vi "WLAN_FrameAnalysisV3.vi"(0 "input cluster":cluster{"t0":dbl, "dt":dbl, "Y":cdb[]}, 5 "error in (no error)":errorcluster) -> (3 "SNR dB":dbl, 8 "Modulation parameter LP":T1, 9 "outputbitsHP":i8[](array[numeric]), 10 "SIG valid?":bool, 11 "Frequency offset":dbl, 12 "SNR dB HP":dbl, 13 "SNR dB LP":dbl, 14 "output bits":i8[](array[numeric]), 16 "Modulation parameter":T1, 17 "Constellation":cdb[](graph), 19 "error out":errorcluster)   [LabVIEW 2022 SP3]
panel:
  in  "Expected message HP":string="Critical Dataaaaa\nCritical Dataaaaa\nCritical Dataaaaa\nCritical Dataaaaa\nCritical Dataaaaa"
  in  "Expected message LP":string="Non Critical Data\nNon Critical Data\nNon Critical Data\nNon Critical Data\nNon Critical Data"
  out "SNR Valid?":bool
  out "Noise Power":dbl
  out "Signal Power":dbl
  out "Alpha":u32
  out "subarray":cdb[](array[numeric])
  out "size(s) 6":i32
  out "size(s) 5":i32
  out "size(s) 4":i32
  out "x+y":dbl
  out "Frequency offset(LTF)":dbl
  out "Frequency offset corrected signal 2":cluster{"t0":dbl, "dt":dbl, "Y":dbl[]}(graph)
  out "size(s) 3":i32
  out "size(s) 2":i32
  out "size(s)":i32
  out "Symbol numbers":i32
  out "encoded bit numbers":u32
  out "original bit numbers":u32
  out "Channel Esitimate":dbl[](graph)
  out "Frequency offset corrected signal":cluster{"t0":dbl, "dt":dbl, "Y":dbl[]}(graph)
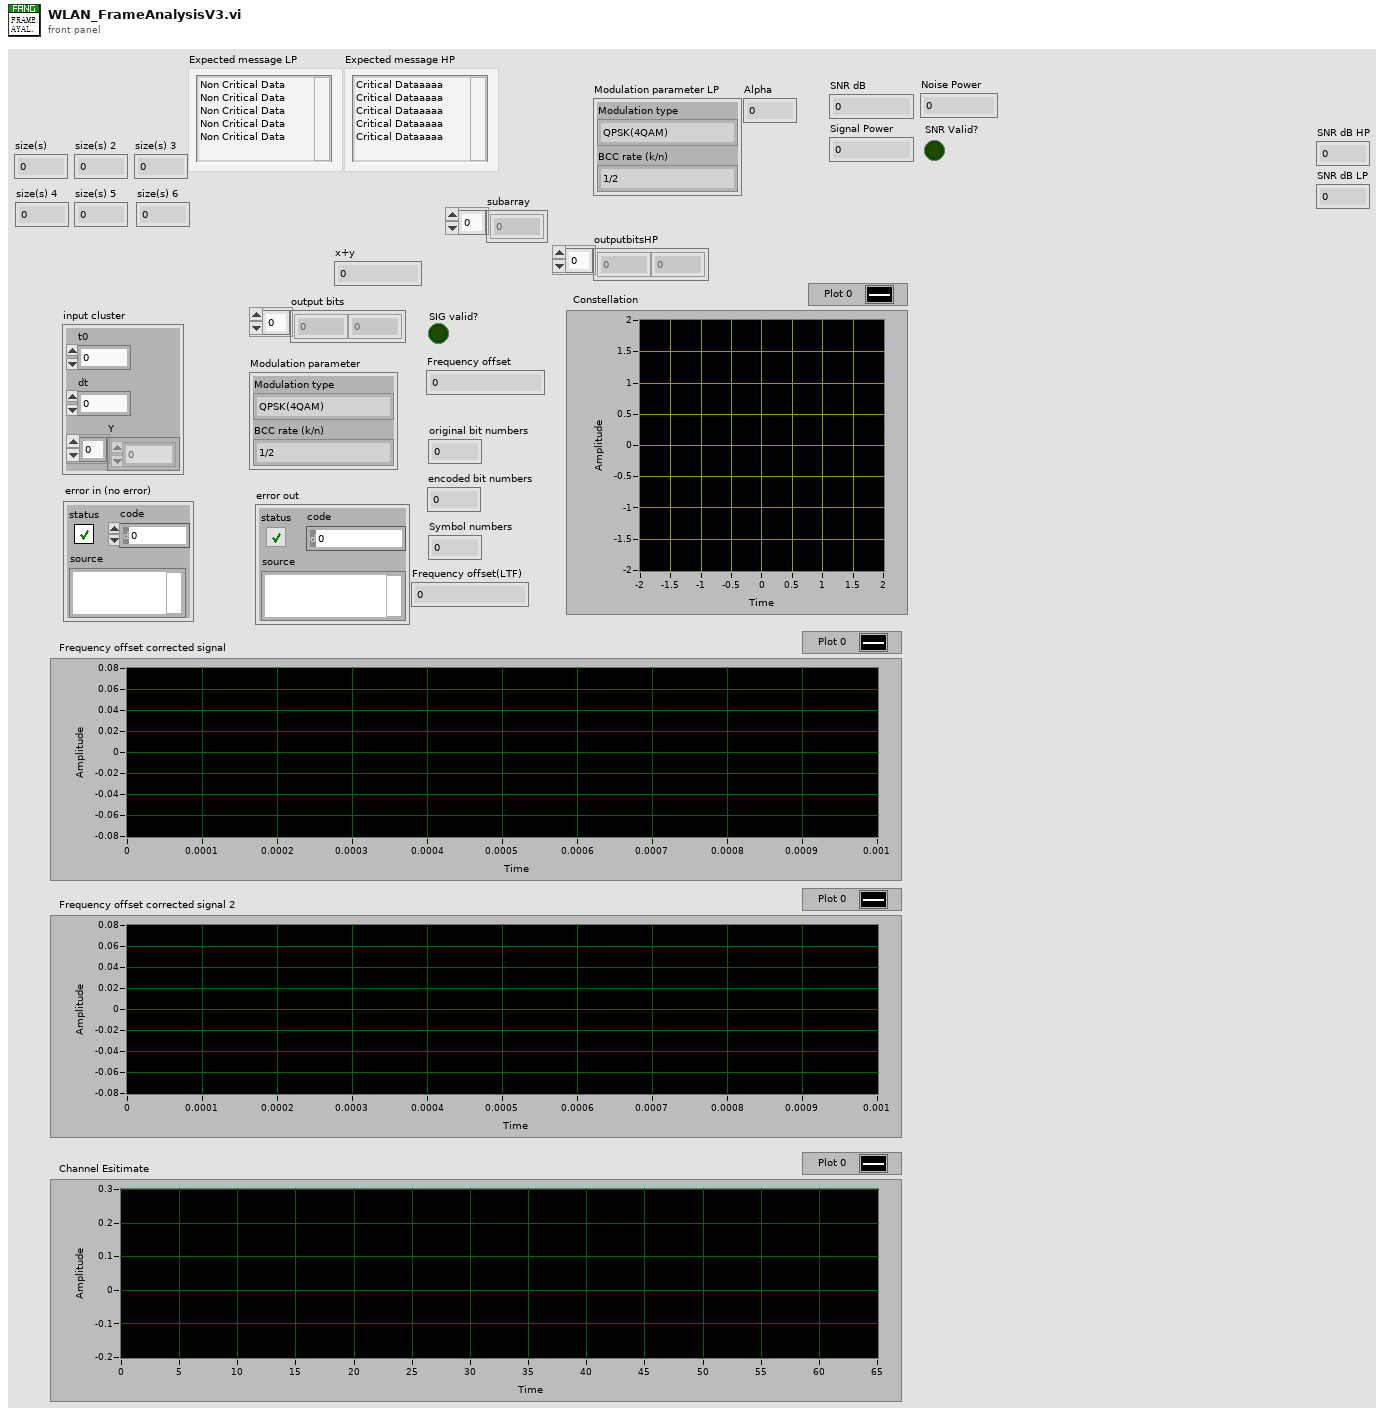
[diagram p1: front panel]
types:
  T1 = cluster{"Modulation type":enum16{"QPSK(4QAM)", "64QAM", "16QAM", "BPSK"}, "BCC rate (k/n)":enum16{"1/2", "2/3", "3/4"}}
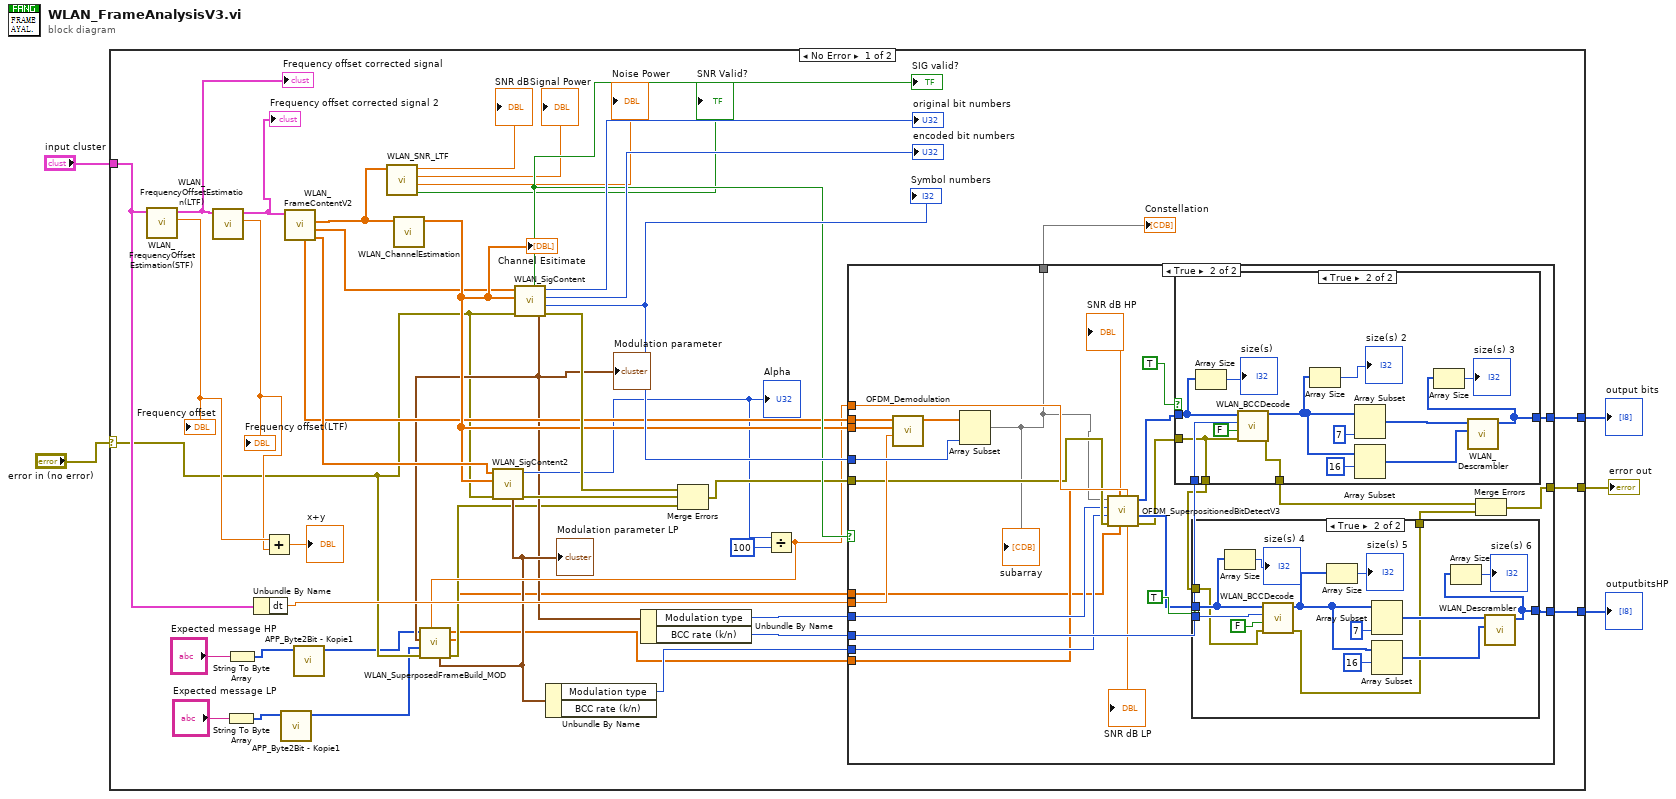
[diagram p0: block diagram]
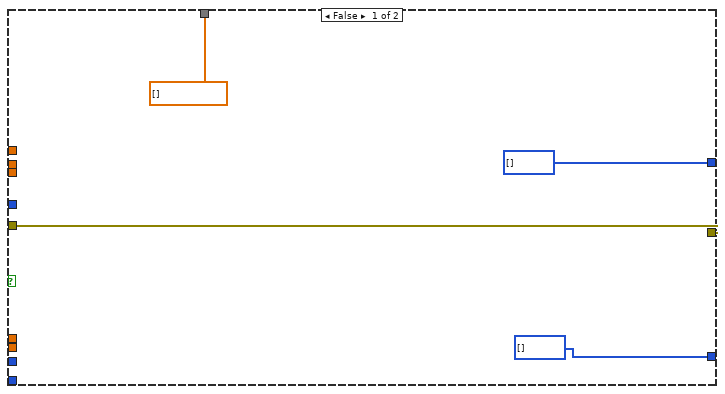
[diagram p2: hidden frame]
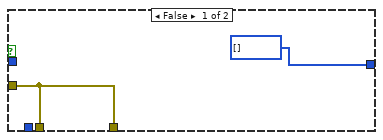
[diagram p3: hidden frame]
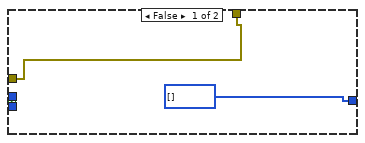
[diagram p4: hidden frame]
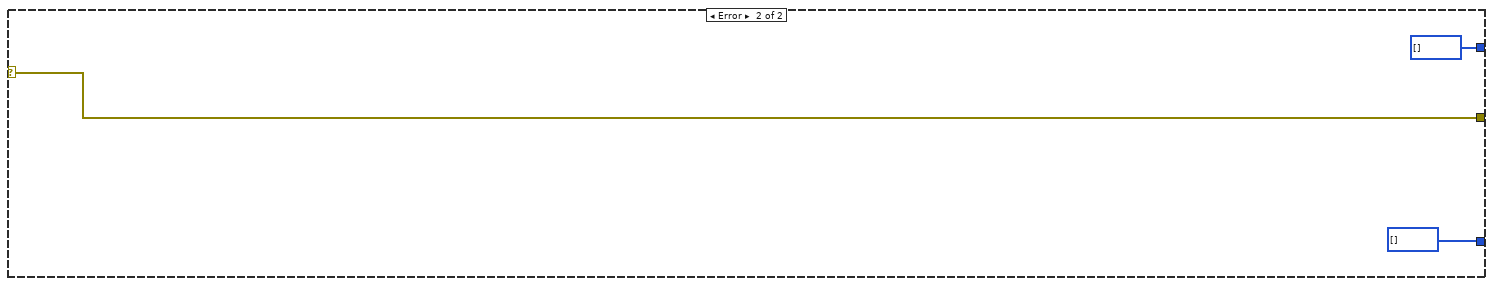
[diagram p5: hidden frame]
diagram:
  n1 = case shown="No Error" "error in (no error)" {
    selector: "error in (no error)" -> [w15 w114]
    tunnel: "input cluster" -> [w37 _]
    tunnel: [w47 w114] -> w4
    tunnel: [w46 i8[] [] ("scrambled bits")] -> w3
    tunnel: [w35 i8[] [] ("scrambled bits")] -> w1
    frame No Error {
      n2 = call "WLAN_FrequencyOffsetEstimation(STF).vi"("output cluster"=w37) -> ("Frequency offset(STF)"=w40:dbl, "output cluster 2"=w41:cluster{"t0":dbl, "dt":dbl, "Y":cdb[]})  [unwired: 8 in]
      "Frequency offset corrected signal" <- w41
      "Frequency offset" <- w40
      n3 = call "WLAN_FrequencyOffsetEstimation(LTF).vi"("input cluster"=w41) -> ("Frequency offset(LTF)"=w39:dbl, "output cluster"=w26:cluster{"t0":dbl, "dt":dbl, "Y":cdb[]})  [unwired: 9 in]
      "Frequency offset corrected signal 2" <- w26
      "Frequency offset(LTF)" <- w39
      n4 = String To Byte Array(string="Expected message LP") -> (unsigned byte array=w9:u8[])
      n5 = String To Byte Array(string="Expected message HP") -> (unsigned byte array=w11:u8[])
      n6 = Unbundle By Name(w37) -> ("dt"=w36:dbl)
      n7 = Add(x=w40, y=w39) -> (x+y=→"x+y":dbl)
      n8 = call "APP_Byte2Bit - Kopie1.vi"("input byte stream"=w9) -> ("output bit stream"=w8:i8[])  [unwired: 10 in]
      n9 = call "WLAN_FrameContentV2.vi"("Input cluster"=w26) -> ("SIG 2"=w30:cdb[], "SIG"=w28:cdb[], "LTF"=w23:cdb[], "DATA"=w27:cdb[])  [unwired: 6 in, 1 out]
      n10 = call "APP_Byte2Bit - Kopie1.vi"("input byte stream"=w11) -> ("output bit stream"=w10:i8[])  [unwired: 10 in]
      n11 = call "WLAN_SNR_LTF.vi"("LTF Corrected"=w23) -> ("SNR Valid?"=→"SNR Valid?":bool, "Noise Power"=→"Noise Power":dbl, "Signal Power"=→"Signal Power":dbl, "SNR dB"=→"SNR dB":dbl)  [unwired: 7 in]
      n12 = call "WLAN_ChannelEstimation.vi"("LTF"=w23) -> ("Frequency estimation"=w29:cdb[])  [unwired: 10 in]
      "Channel Esitimate" <- w29
      n13 = call "WLAN_SigContent2.vi"("error in (no error)"=w15, "Frequency channel estimation"=w29, "SIG"=w30) -> ("error out"=w32:errorcluster, "Alpha"=w25:u32, "Modulation parameter LP"=w17:T1)  [unwired: 5 in, 1 out]
      "Modulation parameter LP" <- w17
      "Alpha" <- w25
      n14 = call "WLAN_SigContent.vi"("error in (no error)"=w15, "Frequency channel estimation"=w29, "SIG"=w28) -> ("error out"=w31:errorcluster, "Symbol numbers"=w48:i32, "encoded bit numbers"=→"encoded bit numbers":u32, "original bit numbers"=→"original bit numbers":u32, "Modulation parameter"=w16:T1, "SIG valid?"=w42:bool)  [unwired: 3 in]
      "Modulation parameter" <- w16
      "Symbol numbers" <- w48
      "SIG valid?" <- w42
      n15 = Unbundle By Name(w17) -> ("Modulation type"=w34:enum16{"QPSK(4QAM)", "64QAM", "16QAM", "BPSK"})  [unwired: 1 out]
      n16 = Unbundle By Name(w16) -> ("Modulation type"=w45:enum16{"QPSK(4QAM)", "64QAM", "16QAM", "BPSK"}, "BCC rate (k/n)"=w44:enum16{"1/2", "2/3", "3/4"})
      n17 = Divide(x=w25, y=u32 100) -> (x/y=w18:dbl)
      n18 = call "WLAN_SuperposedFrameBuild_MOD.vi"("Modulation parameter LP"=w17, "Alpha"=w18, "error in (no error)"=w15, "data in 2"=w8, "Modulation parameter HP"=w16, "data in"=w10) -> ("error out"=w14:errorcluster, "symbolsLP"=w6:cdb[], "symbolsHP"=w7:cdb[])  [unwired: 3 in]
      n19 = Merge Errors(w31, w32, w14) -> (w33:errorcluster)
      n20 = case shown="True" w42 {
        tunnel: w27 -> [_ w80]
        tunnel: [w54 w67] -> w47
        tunnel: w29 -> [_ w78]
        tunnel: w33 -> [w54 w62]
        tunnel: w48 -> [_ w77]
        tunnel: w45 -> [_ w60]
        tunnel: [i8[] [] ("scrambled bits") w76] -> w46
        tunnel: w44 -> [_ w74]
        tunnel: [cdb[] [] w59] -> w43
        tunnel: w36 -> [_ w75]
        tunnel: [i8[] [] ("scrambled bits") w73] -> w35
        tunnel: w34 -> [_ w61]
        tunnel: w18 -> [_ w66]
        tunnel: w7 -> [_ w58]
        tunnel: w6 -> [_ w57]
        frame False {
        }
        frame True {
          n21 = call "OFDM_Demodulation.vi"("sampling period"=w75, "Frequency channel estimation"=w78, "Input sequence"=w80) -> ("Output sequence"=w79:cdb[])  [unwired: 8 in]
          n22 = Array Subset(array=w79, length=w77) -> (w59:cdb[])  [unwired: 1 in]
          "subarray" <- w59
          n23 = call "OFDM_SuperpositionedBitDetectV3.vi"("Alpha"=w66, "Input symbolsLP"=w57, "Input symbolsHP"=w58, "error in (no error)"=w62, "Modulation type LP"=w61, "Modulation type"=w60, "Input symbols"=w59) -> ("error out"=w63:errorcluster, "OutputbitsHP"=w64:i8[], "SNR dB HP"=→"SNR dB HP":dbl, "OutputbitsLP"=w65:i8[], "SNR dB LP"=→"SNR dB LP":dbl)
          n24 = case shown="True" TRUE ("need add zeros?") {
            tunnel: w63 -> [w81 w83]
            tunnel: [w81 w96] -> w69
            tunnel: w65 -> [_ w90]
            tunnel: [i8[] [] ("scrambled bits") w85] -> w76
            tunnel: w74 -> [_ w84]
            tunnel: [w81 w83] -> w70
            frame False {
            }
            frame True {
              n25 = Array Size(array=w90) -> (size(s)=→"size(s)":i32)
              n26 = call "WLAN_BCCDecode.vi"("error in (no error)"=w83, "need add zeros?"=FALSE, "BCC rate (k/n)"=w84, "input bit stream"=w90) -> ("error out"=w96:errorcluster, "output bit stream"=w87:i8[])  [unwired: 6 in]
              n27 = Array Size(array=w87) -> (size(s)=→"size(s) 2":i32)
              n28 = Array Subset(array=w87, length=7) -> (w92:i8[])  [unwired: 1 in]
              n29 = Array Subset(array=w87, index=16) -> (w93:i8[])  [unwired: 1 in]
              n30 = call "WLAN_Descrambler.vi"("scrambler initial bits"=w92, "data bits"=w93) -> ("scrambled bits"=w85:i8[])  [unwired: 7 in]
              n31 = Array Size(array=w85) -> (size(s)=→"size(s) 3":i32)
            }
          }
          n32 = case shown="True" TRUE ("need add zeros?") {
            tunnel: w74 -> [_ w111]
            tunnel: w64 -> [_ w110]
            tunnel: [i8[] [] ("scrambled bits") w99] -> w73
            tunnel: w70 -> [w97 w101]
            tunnel: [w97 w100] -> w68
            frame False {
            }
            frame True {
              n33 = Array Size(array=w110) -> (size(s)=→"size(s) 4":i32)
              n34 = call "WLAN_BCCDecode.vi"("error in (no error)"=w101, "need add zeros?"=FALSE, "BCC rate (k/n)"=w111, "input bit stream"=w110) -> ("error out"=w100:errorcluster, "output bit stream"=w107:i8[])  [unwired: 6 in]
              n35 = Array Size(array=w107) -> (size(s)=→"size(s) 5":i32)
              n36 = Array Subset(array=w107, length=7) -> (w103:i8[])  [unwired: 1 in]
              n37 = Array Subset(array=w107, index=16) -> (w104:i8[])  [unwired: 1 in]
              n38 = call "WLAN_Descrambler.vi"("scrambler initial bits"=w103, "data bits"=w104) -> ("scrambled bits"=w99:i8[])  [unwired: 7 in]
              n39 = Array Size(array=w99) -> (size(s)=→"size(s) 6":i32)
            }
          }
          n40 = Merge Errors(w69, w68) -> (w67:errorcluster)
        }
      }
      "Constellation" <- w43
    }
    frame Error {
    }
  }
  "error out" <- w4
  "output bits" <- w3
  "outputbitsHP" <- w1
